vi "Varex-Calibration.vi"(8 "error in":errorcluster, 11 "Calibration in":refnum<class "Calibration.lvclass">) -> (0 "error out":errorcluster, 3 "Calibration out":refnum<class "Calibration.lvclass">)   [LabVIEW 2022 SP3, in "Bontech Calibration.lvlib" / "Calibration.lvclass"]
uses:
  Calibration.lvclass
  Calibration.lvclass/Calibration.ctl
  d077555a-1f94-446a-85b2-7b0ad1c6b4f0.vi
  db90e855-191f-4739-9521-1b2d8c1b96f4.vi
  VarexWrapperLvLib/VarexWrapper.lvlib
panel:
  in  "No of Frames for Calibration":u16=100 min=100 max=10000
  out "GainValid?":bool
  out "OffsetValid?":bool
  in  "Status":string
  in  "Gain":bool
  in  "Offset":bool
  # "Aayvu  Calibration Tool"
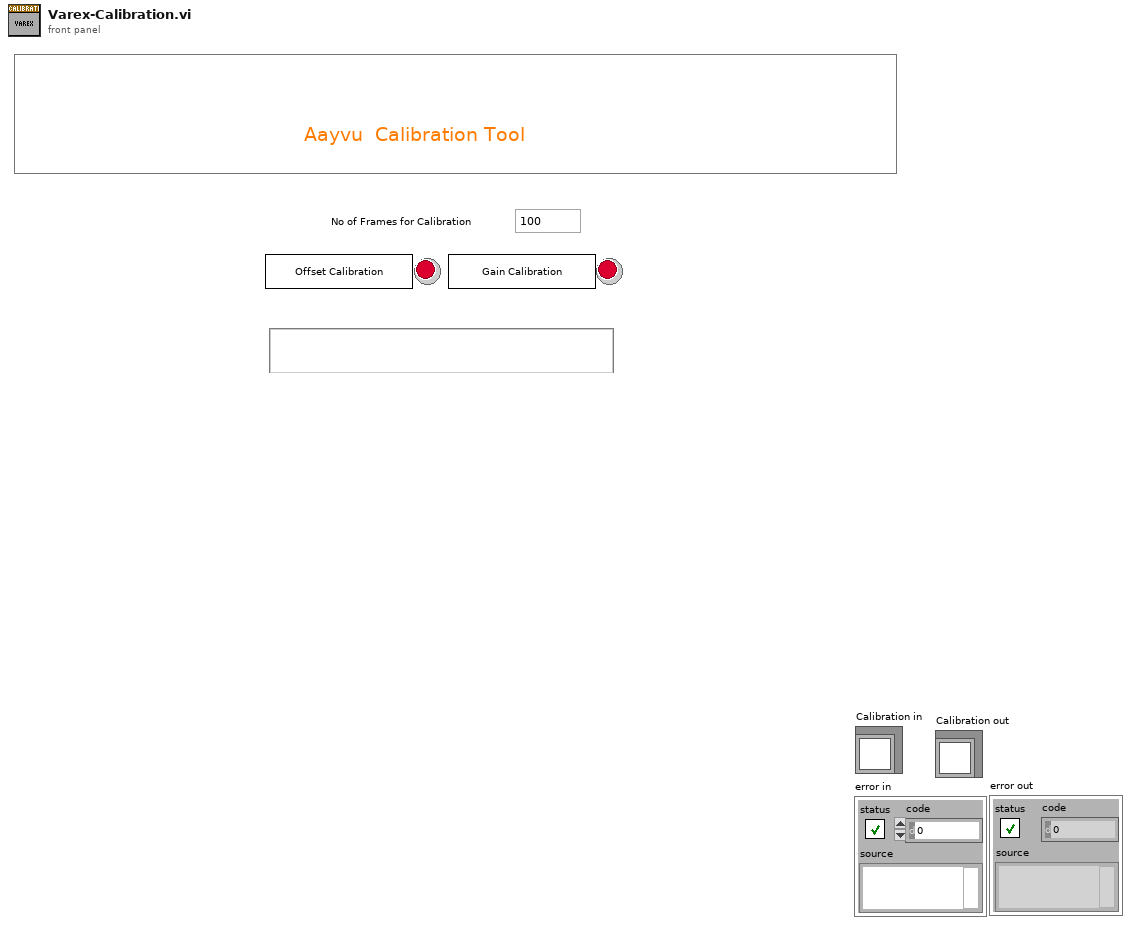
[diagram p1: front panel]
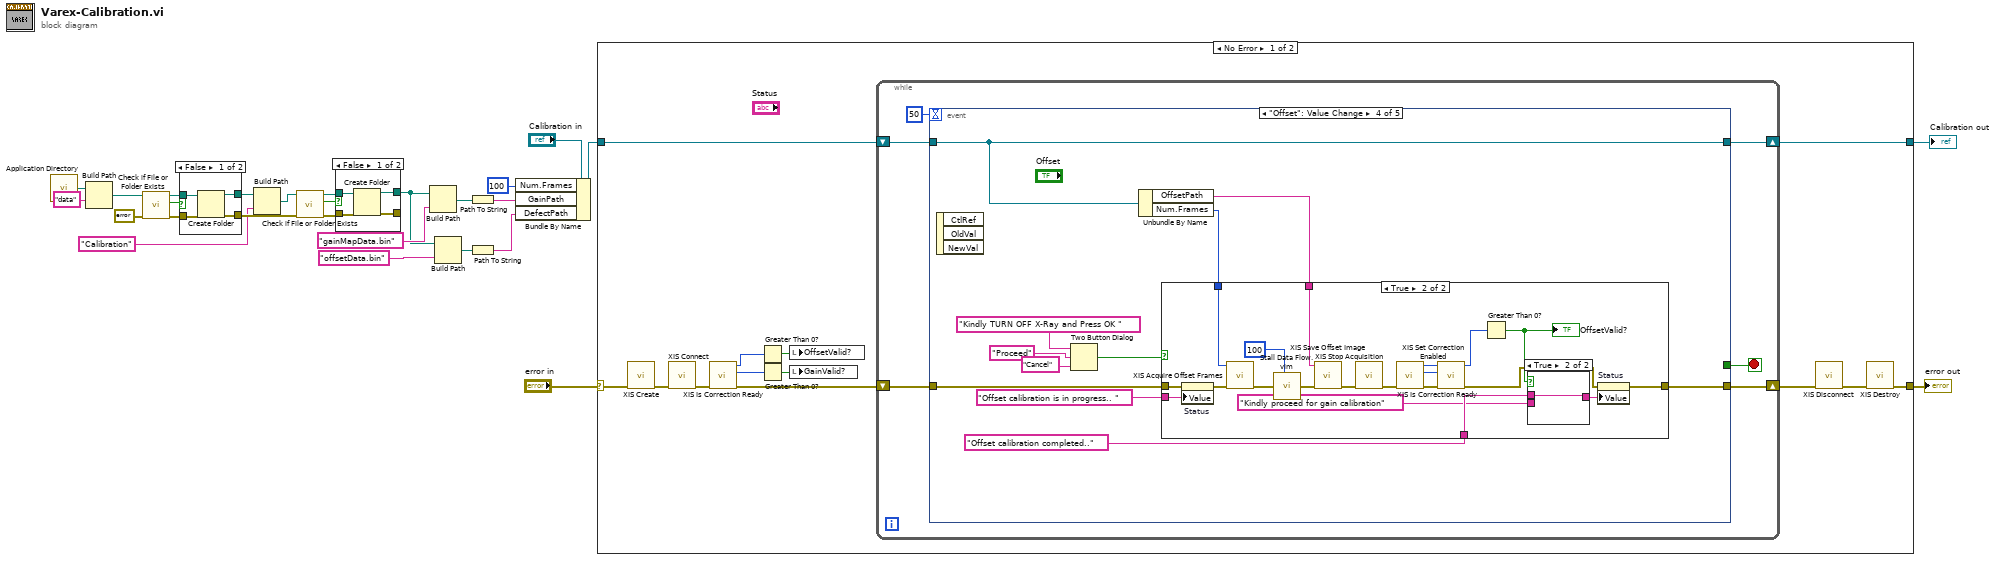
[diagram p0: block diagram]
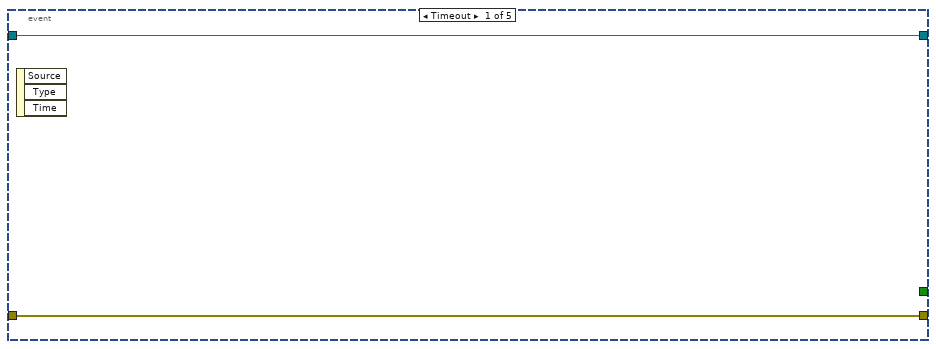
[diagram p4: hidden frame]
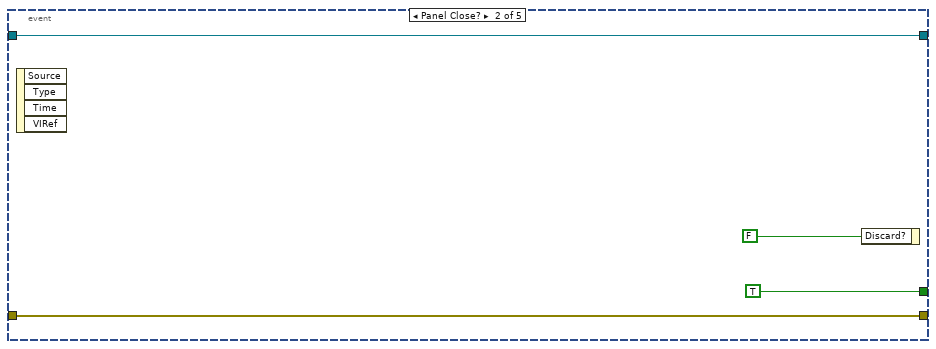
[diagram p5: hidden frame]
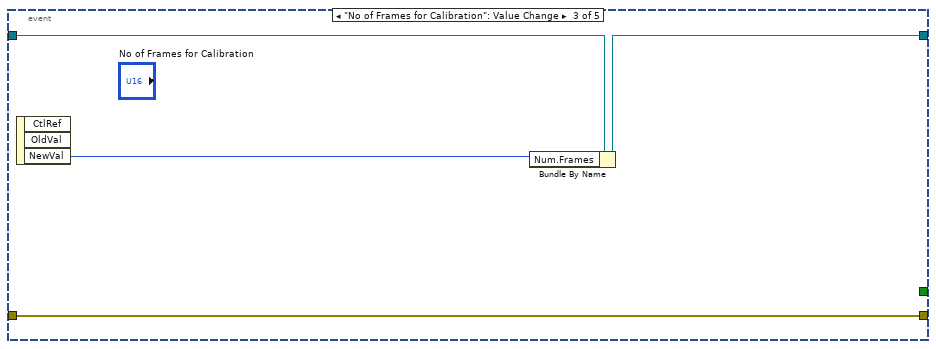
[diagram p6: hidden frame]
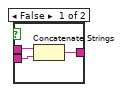
[diagram p8: hidden frame]
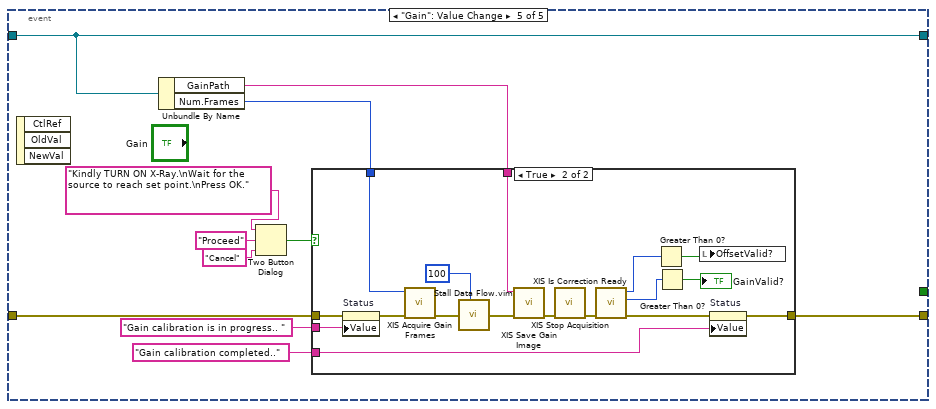
[diagram p9: hidden frame]
diagram:
  n1 = call <vilib>:"Application Directory.vi"() -> ("Application Directory"=w21:path)
  n2 = Build Path(base path=w21, name or relative path="data") -> (appended path=w19:path)
  n3 = call <vilib>:"Check if File or Folder Exists.vi"("error in (no error)"=errorcluster {"status"=FALSE, "code"=0, "source"=""}, "path"=w19) -> ("error out"=w17:errorcluster, "file or folder exists?"=w16:bool, "dup path"=w18:path)  [unwired: 7 in]
  n4 = case shown="False" w16 {
    tunnel: w18 -> [w31 w33]
    tunnel: w17 -> [w30 w32]
    tunnel: [w29 w33] -> w15
    tunnel: [w28 w32] -> w13
    frame False {
      n5 = Create Folder(path (use dialog)=w31, error in=w30) -> (created path=w29:path, error out=w28:errorcluster)  [unwired: 1 in, 1 out]
    }
    frame True {
    }
  }
  n6 = Build Path(base path=w15, name or relative path="Calibration") -> (appended path=w14:path)
  n7 = call <vilib>:"Check if File or Folder Exists.vi"("error in (no error)"=w13, "path"=w14) -> ("error out"=w11:errorcluster, "file or folder exists?"=w10:bool, "dup path"=w9:path)  [unwired: 7 in]
  n8 = case shown="False" w10 {
    tunnel: w9 -> [w37 w39]
    tunnel: w11 -> [w36 w38]
    tunnel: [w35 w39] -> w6
    tunnel: [w34 w38] -> _
    frame False {
      n9 = Create Folder(path (use dialog)=w37, error in=w36) -> (created path=w35:path, error out=w34:errorcluster)  [unwired: 1 in, 1 out]
    }
    frame True {
    }
  }
  n10 = Build Path(base path=w6, name or relative path="gainMapData.bin") -> (appended path=w3:path)
  n11 = Build Path(base path=w6, name or relative path="offsetData.bin") -> (appended path=w4:path)
  n12 = Path To String(path=w3) -> (string=w2:string)
  n13 = Path To String(path=w4) -> (string=w1:string)
  n14 = Bundle By Name(cluster="Calibration in", "Num.Frames"=u16 100 ("Sensor Data.DT/Varex Data.Num.Frames"), "GainPath"=w2, "DefectPath"=w1) -> (w23:refnum<class "Calibration.lvclass">)
  n15 = case shown="No Error" "error in" {
    selector: "error in" -> [w50 w135]
    tunnel: [w40 w135] -> w26
    tunnel: [w51 w134] -> w24
    tunnel: w23 -> [w52 w134]
    frame No Error {
      n16 = call "XIS Create.vi"("error in (no error)"=w50) -> ("error out"=w43:errorcluster)  [unwired: 9 in, 1 out]
      n17 = call "XIS Connect.vi"("error in (no error)"=w43) -> ("error out"=w42:errorcluster)  [unwired: 9 in, 1 out]
      n18 = call "XIS Is Correction Ready.vi"("error in (no error)"=w42) -> ("error out"=w48:errorcluster, "gainReady out"=w46:i32, "offsetReady out"=w47:i32)  [unwired: 7 in, 1 out]
      n19 = Greater Than 0?(x=w47) -> (x > 0?=w45:bool)
      n20 = Greater Than 0?(x=w46) -> (x > 0?=w44:bool)
      n21 = local write "OffsetValid?"(w45) -> ()
      n22 = local write "GainValid?"(w44) -> ()
      n23 = while {
        shift-right: [w57] -> w51
        shift-left: w52 -> [w58]
        shift-right: [w55] -> w49
        shift-left: w48 -> [w56]
        stop <- w53 stop-if-true
        n24 = event shown="[3] \"Offset\": Value Change" {
          selector: _ -> [_ _ _ _ _]
          dyn-events: _ -> [_ _ _ _ _]
          timeout: 50 -> [_ _ _ _ _]
          tunnel: w58 -> [w60 w64 w68 w78 w113]
          tunnel: [w60 w64 w66 w78 w113] -> w57
          tunnel: [w59 w63 w67 w76 w114] -> w55
          tunnel: w56 -> [w59 w63 w67 w79 w115]
          tunnel: [_ TRUE _ _ _] -> w53
          event Timeout {
            n25 = event-data() -> ()  [unwired: 1 in, 3 out]
          }
          event Panel Close? {
            n26 = event-data() -> ()  [unwired: 1 in, 4 out]
            n27 = event-data("Discard?"=FALSE) -> ()  [unwired: 1 in, 1 out]
          }
          event "No of Frames for Calibration": Value Change {
            n28 = event-data() -> ("NewVal"=w65:u16)  [unwired: 1 in, 2 out]
            n29 = Bundle By Name(cluster=w68, "Num.Frames"=w65) -> (w66:refnum<class "Calibration.lvclass">)
          }
          event "Offset": Value Change {
            n30 = event-data() -> ()  [unwired: 1 in, 3 out]
            n31 = Two Button Dialog(message="Kindly TURN OFF X-Ray and Press OK " ("Value"), 1:"Cancel" ("F button name (\"Cancel\")"), 2:"Proceed" ("T button name (\"OK\")")) -> (T button?=w70:bool)
            n32 = Unbundle By Name(w78) -> ("OffsetPath"=w69:string, "Num.Frames"=w77:u16)
            n33 = case shown="True" w70 {
              tunnel: w79 -> [w80 w100]
              tunnel: w77 -> [_ w94]
              tunnel: [w80 w91] -> w76
              tunnel: "Offset calibration completed.." ("Value") -> [_ w90]
              tunnel: "Offset calibration is in progress.. " ("Value") -> [_ w87]
              tunnel: w69 -> [_ w86]
              frame False {
              }
              frame True {
                n34 = property on="Status" class="Str"(error in=w100, "Value"=w87) -> (error out=w92:errorcluster)  [unwired: 1 in, 1 out]
                n35 = call "XIS Acquire Offset Frames.vi"("error in (no error)"=w92, "numFrames"=w94) -> ("error out"=w99:errorcluster)  [unwired: 8 in, 1 out]
                n36 = call "Stall Data Flow.vim"("value in"=w99, "milliseconds to wait"=u32 100) -> ("value out"=w98:errorcluster)  [unwired: 1 out]
                n37 = call "XIS Save Offset Image.vi"("error in (no error)"=w98, "filePath"=w86) -> ("error out"=w97:errorcluster)  [unwired: 8 in, 1 out]
                n38 = call "XIS Stop Acquisition.vi"("error in (no error)"=w97) -> ("error out"=w96:errorcluster)  [unwired: 9 in, 1 out]
                n39 = call "XIS Is Correction Ready.vi"("error in (no error)"=w96) -> ("error out"=w95:errorcluster, "gainReady out"=w83:i32, "offsetReady out"=w84:i32)  [unwired: 7 in, 1 out]
                n40 = call "XIS Set Correction Enabled.vi"("error in (no error)"=w95, "enableGain"=w83, "enableOffset"=w84) -> ("error out"=w85:errorcluster, "function return"=w82:i32)  [unwired: 7 in]
                n41 = Greater Than 0?(x=w82) -> (x > 0?=w81:bool)
                "OffsetValid?" <- w81
                n42 = case shown="True" w81 {
                  tunnel: w90 -> [w103 w104]
                  tunnel: [w102 w104] -> w89
                  tunnel: "Kindly proceed for gain calibration" ("Value") -> [w101 _]
                  frame False {
                    n43 = Concatenate Strings(w103, w101) -> (w102:string)
                  }
                  frame True {
                  }
                }
                n44 = property on="Status" class="Str"(error in=w85, "Value"=w89) -> (error out=w91:errorcluster)  [unwired: 1 in, 1 out]
              }
            }
          }
          event "Gain": Value Change {
            n45 = event-data() -> ()  [unwired: 1 in, 3 out]
            n46 = Unbundle By Name(w113) -> ("GainPath"=w105:string, "Num.Frames"=w112:u16)
            n47 = Two Button Dialog(message="Kindly TURN ON X-Ray.\nWait for the source to reach set point.\nPress OK." ("Value"), 1:"Cancel" ("F button name (\"Cancel\")"), 2:"Proceed" ("T button name (\"OK\")")) -> (T button?=w109:bool)
            n48 = case shown="True" w109 {
              tunnel: w115 -> [w116 w133]
              tunnel: [w116 w123] -> w114
              tunnel: w112 -> [_ w129]
              tunnel: "Gain calibration is in progress.. " ("Value") -> [_ w122]
              tunnel: "Gain calibration completed.." ("Value") -> [_ w121]
              tunnel: w105 -> [_ w120]
              frame False {
              }
              frame True {
                n49 = property on="Status" class="Str"(error in=w133, "Value"=w122) -> (error out=w124:errorcluster)  [unwired: 1 in, 1 out]
                n50 = call "XIS Acquire Gain Frames.vi"("error in (no error)"=w124, "numFrames"=w129) -> ("error out"=w132:errorcluster)  [unwired: 8 in, 1 out]
                n51 = call "Stall Data Flow.vim"("value in"=w132, "milliseconds to wait"=u32 100) -> ("value out"=w118:errorcluster)  [unwired: 1 out]
                n52 = call "XIS Save Gain Image.vi"("error in (no error)"=w118, "filePath"=w120) -> ("error out"=w131:errorcluster)  [unwired: 8 in, 1 out]
                n53 = call "XIS Stop Acquisition.vi"("error in (no error)"=w131) -> ("error out"=w117:errorcluster)  [unwired: 9 in, 1 out]
                n54 = call "XIS Is Correction Ready.vi"("error in (no error)"=w117) -> ("error out"=w130:errorcluster, "gainReady out"=w126:i32, "offsetReady out"=w128:i32)  [unwired: 7 in, 1 out]
                n55 = Greater Than 0?(x=w128) -> (x > 0?=w119:bool)
                n56 = Greater Than 0?(x=w126) -> (x > 0?=→"GainValid?":bool)
                n57 = local write "OffsetValid?"(w119) -> ()
                n58 = property on="Status" class="Str"(error in=w130, "Value"=w121) -> (error out=w123:errorcluster)  [unwired: 1 in, 1 out]
              }
            }
          }
        }
      }
      n59 = call "XIS Disconnect.vi"("error in (no error)"=w49) -> ("error out"=w41:errorcluster)  [unwired: 9 in, 1 out]
      n60 = call "XIS Destroy.vi"("error in (no error)"=w41) -> ("error out"=w40:errorcluster)  [unwired: 9 in, 1 out]
    }
    frame Error {
    }
  }
  "error out" <- w26
  "Calibration out" <- w24
